vi "Update Method Accessors.vi"(7 "Library":refnum<vi>, 8 "error in (no error)":errorcluster, 10 "RPC Method Parameters":T1, 11 "Server class in":refnum<vi>) -> (0 "error out":errorcluster, 3 "Server class out":refnum<vi>)   [LabVIEW 2019, in "gRPC Template Creation Utility.lvlib"]
uses:
  gRPC Template Creation Utility.lvlib
  TypeDefs/RPC Method Parameters.ctl
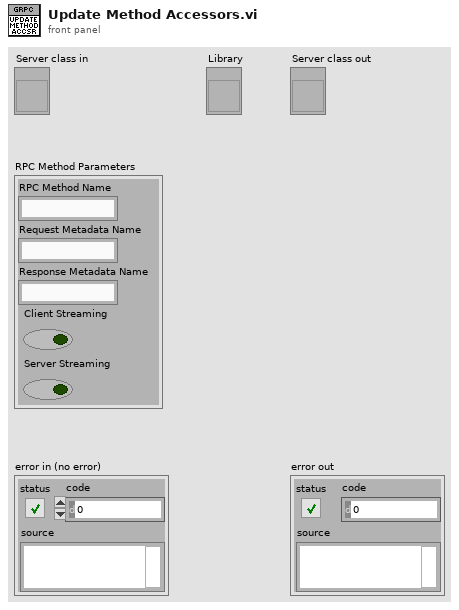
[diagram p1: front panel]
types:
  T1 = typedef "gRPC Template Creation Utility.lvlib/RPC Method Parameters.ctl" = cluster{"RPC Method Name":string, "Request Metadata Name":string, "Response Metadata Name":string, "Client Streaming":bool, "Server Streaming":bool}
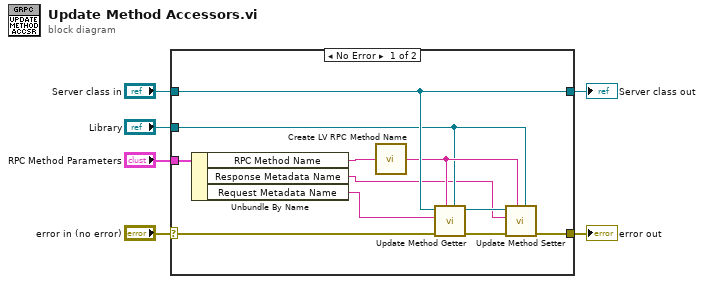
[diagram p0: block diagram]
diagram:
  n1 = case shown="No Error" "error in (no error)" {
    selector: "error in (no error)" -> [w16 w18]
    tunnel: "RPC Method Parameters" -> [w17 _]
    tunnel: "Server class in" -> [w12 w19]
    tunnel: [w12 w19] -> w3
    tunnel: [w13 w18] -> w2
    tunnel: "Library" -> [w9 _]
    frame No Error {
      n2 = Unbundle By Name(w17) -> ("RPC Method Name"=w11:string, "Response Metadata Name"=w7:string, "Request Metadata Name"=w8:string)
      n3 = call "Create LV RPC Method Name.vi"("Proto Parser RPC Method Name in"=w11) -> ("LV RPC Method Name out"=w10:string)
      n4 = call "Update Method Getter.vi"("Library"=w9, "RPC Method Name"=w10, "error in (no error)"=w16, "Request Metadata Name"=w8, "Server class in"=w12) -> ("error out"=w15:errorcluster, "Server class out"=w14:refnum<vi>)  [unwired: 5 in]
      n5 = call "Update Method Setter.vi"("Library"=w9, "RPC Method Name"=w10, "error in (no error)"=w15, "Response Metadata Name"=w7, "Server class in"=w14) -> ("error out"=w13:errorcluster)  [unwired: 5 in, 1 out]
    }
    frame Error {
    }
  }
  "error out" <- w2
  "Server class out" <- w3
